vi "Init AS7431.vi"(8 "error in (no error)":errorcluster, 11 "AS7431 Light Spectrum in":refnum<class "AS7431 11 Ch Light Spectrum Sensor.lvclass">) -> (0 "error out":errorcluster, 3 "AS7431 Light Spectrum out":refnum<class "AS7431 11 Ch Light Spectrum Sensor.lvclass">)   [LabVIEW 2020, in "CTI-Peripheral.lvlib" / "AS7431 11 Ch Light Spectrum Sensor.lvclass"]
uses:
  AS7431 11 Ch Light Spectrum Sensor.lvclass
  AS7431 11 Ch Light Spectrum Sensor.lvclass/AS7431 11 Ch Light Spectrum Sensor.ctl
  CTI/I2C Connection/I2C Connection.lvclass/I2C Connection.ctl
  CTI/Session/I2C Write Data.vi
  CTI/Session/I2C Read Data.vi
  CTI/I2C Connection/I2C Connection.lvclass
panel:
  out "Chip ID":string
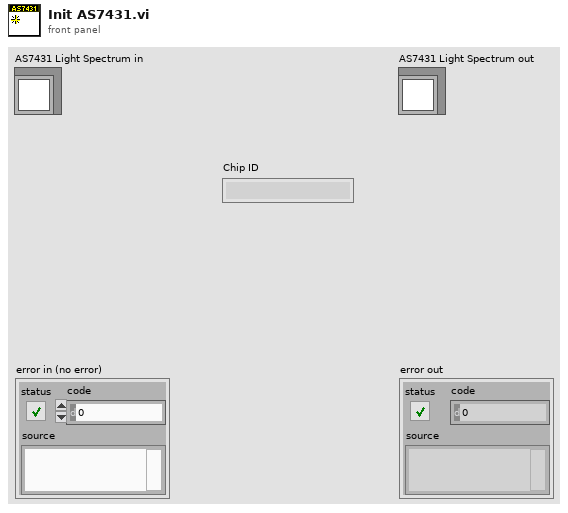
[diagram p1: front panel]
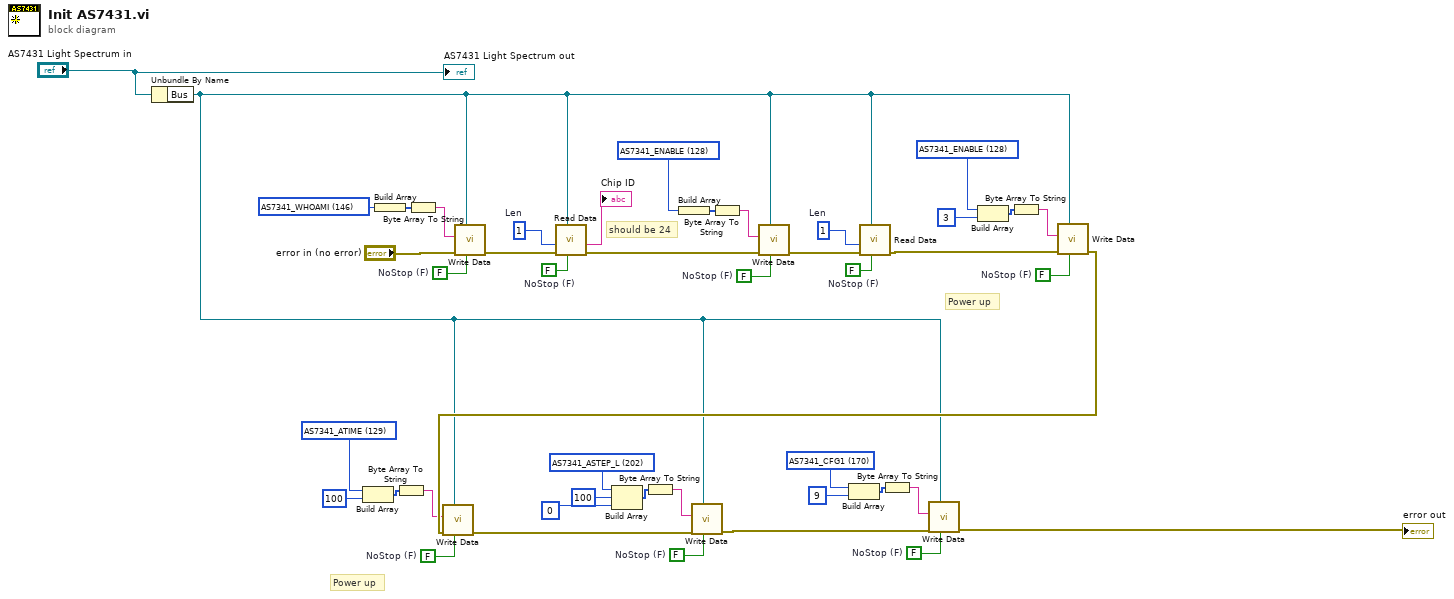
[diagram p0: block diagram]
diagram:
  w4 = FALSE  # NoStop (F)
  w7 = u16 170 items=["AS7341_I2CADDR_DEFAULT"=57, "AS7341_CHIP_ID"=9, "AS7341_WHOAMI"=146, "AS7341_CONFIG"=112, "AS7341_GPIO"=115, "AS7341_LED"=116, "AS7341_ENABLE"=128, "AS7341_ATIME"=129, "AS7341_SP_LOW_TH_L"=132, "AS7341_SP_LOW_TH_H"=133, "AS7341_SP_HIGH_TH_L"=134, "AS7341_SP_HIGH_TH_H"=135, "AS7341_STATUS"=147, "AS7341_ASTATUS_"=148, "AS7341_CH0_DATA_L"=149, "AS7341_CH0_DATA_H"=150, "AS7341_CH1_DATA_L"=151, "AS7341_CH1_DATA_H"=152, "AS7341_CH2_DATA_L"=153, "AS7341_CH2_DATA_H"=154, "AS7341_CH3_DATA_L"=155, "AS7341_CH3_DATA_H"=156, "AS7341_CH4_DATA_L"=157, "AS7341_CH4_DATA_H"=158, "AS7341_CH5_DATA_L"=159, "AS7341_CH5_DATA_H"=160, "AS7341_STATUS2"=163, "AS7341_STATUS3"=164, "AS7341_CFG0"=169, "AS7341_CFG1"=170, "AS7341_CFG6"=175, "AS7341_CFG9"=178, "AS7341_CFG12"=181, "AS7341_PERS"=189, "AS7341_GPIO2"=190, "AS7341_ASTEP_L"=202, "AS7341_ASTEP_H"=203, "AS7341_FD_TIME1"=216, "AS7341_FD_TIME2"=218, "AS7341_FD_STATUS"=219, "AS7341_INTENAB"=249, "AS7341_CONTROL"=250] ("Registers")
  w14 = FALSE  # NoStop (F)
  w11 = u16 202 items=["AS7341_I2CADDR_DEFAULT"=57, "AS7341_CHIP_ID"=9, "AS7341_WHOAMI"=146, "AS7341_CONFIG"=112, "AS7341_GPIO"=115, "AS7341_LED"=116, "AS7341_ENABLE"=128, "AS7341_ATIME"=129, "AS7341_SP_LOW_TH_L"=132, "AS7341_SP_LOW_TH_H"=133, "AS7341_SP_HIGH_TH_L"=134, "AS7341_SP_HIGH_TH_H"=135, "AS7341_STATUS"=147, "AS7341_ASTATUS_"=148, "AS7341_CH0_DATA_L"=149, "AS7341_CH0_DATA_H"=150, "AS7341_CH1_DATA_L"=151, "AS7341_CH1_DATA_H"=152, "AS7341_CH2_DATA_L"=153, "AS7341_CH2_DATA_H"=154, "AS7341_CH3_DATA_L"=155, "AS7341_CH3_DATA_H"=156, "AS7341_CH4_DATA_L"=157, "AS7341_CH4_DATA_H"=158, "AS7341_CH5_DATA_L"=159, "AS7341_CH5_DATA_H"=160, "AS7341_STATUS2"=163, "AS7341_STATUS3"=164, "AS7341_CFG0"=169, "AS7341_CFG1"=170, "AS7341_CFG6"=175, "AS7341_CFG9"=178, "AS7341_CFG12"=181, "AS7341_PERS"=189, "AS7341_GPIO2"=190, "AS7341_ASTEP_L"=202, "AS7341_ASTEP_H"=203, "AS7341_FD_TIME1"=216, "AS7341_FD_TIME2"=218, "AS7341_FD_STATUS"=219, "AS7341_INTENAB"=249, "AS7341_CONTROL"=250] ("Registers")
  w15 = FALSE  # NoStop (F)
  w19 = u16 129 items=["AS7341_I2CADDR_DEFAULT"=57, "AS7341_CHIP_ID"=9, "AS7341_WHOAMI"=146, "AS7341_CONFIG"=112, "AS7341_GPIO"=115, "AS7341_LED"=116, "AS7341_ENABLE"=128, "AS7341_ATIME"=129, "AS7341_SP_LOW_TH_L"=132, "AS7341_SP_LOW_TH_H"=133, "AS7341_SP_HIGH_TH_L"=134, "AS7341_SP_HIGH_TH_H"=135, "AS7341_STATUS"=147, "AS7341_ASTATUS_"=148, "AS7341_CH0_DATA_L"=149, "AS7341_CH0_DATA_H"=150, "AS7341_CH1_DATA_L"=151, "AS7341_CH1_DATA_H"=152, "AS7341_CH2_DATA_L"=153, "AS7341_CH2_DATA_H"=154, "AS7341_CH3_DATA_L"=155, "AS7341_CH3_DATA_H"=156, "AS7341_CH4_DATA_L"=157, "AS7341_CH4_DATA_H"=158, "AS7341_CH5_DATA_L"=159, "AS7341_CH5_DATA_H"=160, "AS7341_STATUS2"=163, "AS7341_STATUS3"=164, "AS7341_CFG0"=169, "AS7341_CFG1"=170, "AS7341_CFG6"=175, "AS7341_CFG9"=178, "AS7341_CFG12"=181, "AS7341_PERS"=189, "AS7341_GPIO2"=190, "AS7341_ASTEP_L"=202, "AS7341_ASTEP_H"=203, "AS7341_FD_TIME1"=216, "AS7341_FD_TIME2"=218, "AS7341_FD_STATUS"=219, "AS7341_INTENAB"=249, "AS7341_CONTROL"=250] ("Registers")
  w27 = FALSE  # NoStop (F)
  w22 = u16 128 items=["AS7341_I2CADDR_DEFAULT"=57, "AS7341_CHIP_ID"=9, "AS7341_WHOAMI"=146, "AS7341_CONFIG"=112, "AS7341_GPIO"=115, "AS7341_LED"=116, "AS7341_ENABLE"=128, "AS7341_ATIME"=129, "AS7341_SP_LOW_TH_L"=132, "AS7341_SP_LOW_TH_H"=133, "AS7341_SP_HIGH_TH_L"=134, "AS7341_SP_HIGH_TH_H"=135, "AS7341_STATUS"=147, "AS7341_ASTATUS_"=148, "AS7341_CH0_DATA_L"=149, "AS7341_CH0_DATA_H"=150, "AS7341_CH1_DATA_L"=151, "AS7341_CH1_DATA_H"=152, "AS7341_CH2_DATA_L"=153, "AS7341_CH2_DATA_H"=154, "AS7341_CH3_DATA_L"=155, "AS7341_CH3_DATA_H"=156, "AS7341_CH4_DATA_L"=157, "AS7341_CH4_DATA_H"=158, "AS7341_CH5_DATA_L"=159, "AS7341_CH5_DATA_H"=160, "AS7341_STATUS2"=163, "AS7341_STATUS3"=164, "AS7341_CFG0"=169, "AS7341_CFG1"=170, "AS7341_CFG6"=175, "AS7341_CFG9"=178, "AS7341_CFG12"=181, "AS7341_PERS"=189, "AS7341_GPIO2"=190, "AS7341_ASTEP_L"=202, "AS7341_ASTEP_H"=203, "AS7341_FD_TIME1"=216, "AS7341_FD_TIME2"=218, "AS7341_FD_STATUS"=219, "AS7341_INTENAB"=249, "AS7341_CONTROL"=250] ("Registers")
  w34 = FALSE  # NoStop (F)
  w33 = u8 1  # Len
  w30 = FALSE  # NoStop (F)
  w38 = FALSE  # NoStop (F)
  w39 = u8 1  # Len
  w41 = u16 146 items=["AS7341_I2CADDR_DEFAULT"=57, "AS7341_CHIP_ID"=9, "AS7341_WHOAMI"=146, "AS7341_CONFIG"=112, "AS7341_GPIO"=115, "AS7341_LED"=116, "AS7341_ENABLE"=128, "AS7341_ATIME"=129, "AS7341_SP_LOW_TH_L"=132, "AS7341_SP_LOW_TH_H"=133, "AS7341_SP_HIGH_TH_L"=134, "AS7341_SP_HIGH_TH_H"=135, "AS7341_STATUS"=147, "AS7341_ASTATUS_"=148, "AS7341_CH0_DATA_L"=149, "AS7341_CH0_DATA_H"=150, "AS7341_CH1_DATA_L"=151, "AS7341_CH1_DATA_H"=152, "AS7341_CH2_DATA_L"=153, "AS7341_CH2_DATA_H"=154, "AS7341_CH3_DATA_L"=155, "AS7341_CH3_DATA_H"=156, "AS7341_CH4_DATA_L"=157, "AS7341_CH4_DATA_H"=158, "AS7341_CH5_DATA_L"=159, "AS7341_CH5_DATA_H"=160, "AS7341_STATUS2"=163, "AS7341_STATUS3"=164, "AS7341_CFG0"=169, "AS7341_CFG1"=170, "AS7341_CFG6"=175, "AS7341_CFG9"=178, "AS7341_CFG12"=181, "AS7341_PERS"=189, "AS7341_GPIO2"=190, "AS7341_ASTEP_L"=202, "AS7341_ASTEP_H"=203, "AS7341_FD_TIME1"=216, "AS7341_FD_TIME2"=218, "AS7341_FD_STATUS"=219, "AS7341_INTENAB"=249, "AS7341_CONTROL"=250] ("Registers")
  w28 = u16 128 items=["AS7341_I2CADDR_DEFAULT"=57, "AS7341_CHIP_ID"=9, "AS7341_WHOAMI"=146, "AS7341_CONFIG"=112, "AS7341_GPIO"=115, "AS7341_LED"=116, "AS7341_ENABLE"=128, "AS7341_ATIME"=129, "AS7341_SP_LOW_TH_L"=132, "AS7341_SP_LOW_TH_H"=133, "AS7341_SP_HIGH_TH_L"=134, "AS7341_SP_HIGH_TH_H"=135, "AS7341_STATUS"=147, "AS7341_ASTATUS_"=148, "AS7341_CH0_DATA_L"=149, "AS7341_CH0_DATA_H"=150, "AS7341_CH1_DATA_L"=151, "AS7341_CH1_DATA_H"=152, "AS7341_CH2_DATA_L"=153, "AS7341_CH2_DATA_H"=154, "AS7341_CH3_DATA_L"=155, "AS7341_CH3_DATA_H"=156, "AS7341_CH4_DATA_L"=157, "AS7341_CH4_DATA_H"=158, "AS7341_CH5_DATA_L"=159, "AS7341_CH5_DATA_H"=160, "AS7341_STATUS2"=163, "AS7341_STATUS3"=164, "AS7341_CFG0"=169, "AS7341_CFG1"=170, "AS7341_CFG6"=175, "AS7341_CFG9"=178, "AS7341_CFG12"=181, "AS7341_PERS"=189, "AS7341_GPIO2"=190, "AS7341_ASTEP_L"=202, "AS7341_ASTEP_H"=203, "AS7341_FD_TIME1"=216, "AS7341_FD_TIME2"=218, "AS7341_FD_STATUS"=219, "AS7341_INTENAB"=249, "AS7341_CONTROL"=250] ("Registers")
  w44 = FALSE  # NoStop (F)
  # "Power up"
  # "Power up"
  # "should be 24"
  n1 = Unbundle By Name("AS7431 Light Spectrum in") -> ("Bus"=w2:refnum<class "I2C Connection.lvclass">)
  n2 = Build Array(w19, 100) -> (w17:i32[])
  n3 = Build Array(w41) -> (w40:u16[])
  n4 = Byte Array To String(unsigned byte array=w17) -> (string=w16:string)
  n5 = Byte Array To String(unsigned byte array=w40) -> (string=w43:string)
  n6 = call "Write Data.vi"("NoStop (F)"=w44, "I2C Connection"=w2, "error in (no error)"="error in (no error)", "Data"=w43) -> ("error out"=w36:errorcluster)  [unwired: 7 in]
  n7 = call "Read Data.vi"("NoStop (F)"=w38, "I2C Connection"=w2, "error in (no error)"=w36, "Len"=w39) -> ("error out"=w29:errorcluster, "Data"=→"Chip ID":string)  [unwired: 6 in]
  n8 = Build Array(w11, 100, 0) -> (w12:i32[])
  n9 = Byte Array To String(unsigned byte array=w12) -> (string=w13:string)
  n10 = Build Array(w28) -> (w32:u16[])
  n11 = Byte Array To String(unsigned byte array=w32) -> (string=w31:string)
  n12 = call "Write Data.vi"("NoStop (F)"=w30, "I2C Connection"=w2, "error in (no error)"=w29, "Data"=w31) -> ("error out"=w35:errorcluster)  [unwired: 7 in]
  n13 = Build Array(w7, 9) -> (w6:i32[])
  n14 = call "Read Data.vi"("NoStop (F)"=w34, "I2C Connection"=w2, "error in (no error)"=w35, "Len"=w33) -> ("error out"=w23:errorcluster)  [unwired: 6 in, 1 out]
  n15 = Byte Array To String(unsigned byte array=w6) -> (string=w5:string)
  n16 = Build Array(w22, 3) -> (w25:i32[])
  n17 = Byte Array To String(unsigned byte array=w25) -> (string=w26:string)
  n18 = call "Write Data.vi"("NoStop (F)"=w27, "I2C Connection"=w2, "error in (no error)"=w23, "Data"=w26) -> ("error out"=w24:errorcluster)  [unwired: 7 in]
  n19 = call "Write Data.vi"("NoStop (F)"=w15, "I2C Connection"=w2, "error in (no error)"=w24, "Data"=w16) -> ("error out"=w18:errorcluster)  [unwired: 7 in]
  n20 = call "Write Data.vi"("NoStop (F)"=w14, "I2C Connection"=w2, "error in (no error)"=w18, "Data"=w13) -> ("error out"=w3:errorcluster)  [unwired: 7 in]
  n21 = call "Write Data.vi"("NoStop (F)"=w4, "I2C Connection"=w2, "error in (no error)"=w3, "Data"=w5) -> ("error out"=→"error out":errorcluster)  [unwired: 7 in]
  "AS7431 Light Spectrum out" <- "AS7431 Light Spectrum in"
